vi "[ex ce]_Array - Access 1D Array elements.vi"() -> ()   [LabVIEW 2021]
doc: "<B>Example for CalcExpress script syntax</B>\n\n<B>The VI demonstrates various methods of accessing elements in 1D array</B>\n\nThis example demonstrates a use of Index Arrays and Index Ranges to perform array indexing. IndexRange feature lets you specify a sequential index subset of an array dimension. Index Array can be used to specify an arbitrary set of indeces.\n\nTo provide the Index Range feature, CalcExpress supports IndexRange Operator, IndexRange Symbols and a few IndexRange Functions. Despite they have different syntax, they have the similar functionality, so you can use any of them to specify range of indeces. In general, IndexRange symbols and functions can be convenient if you need to specify entire dimension, and IndexRange Operator can be convenient if you need to specify a sequential index subset.\n\n::: CalcExpress Toolkit :::\nCopyright (c) 2000-2026 Konstantin Shifershteyn. All rights reserved."
panel:
  in  "stop":bool
  in  "calc":bool
  in  "Expression":string
  in  "comments":string="This example demonstrates a use of Index Arrays and Index Ranges to perform array indexing. IndexRange feature lets you specify a sequential index subset of an array dimension. Index Array can be used to specify an arbitrary set of indeces.\n\nTo provide the Index Range feature, CalcExpress supports IndexRange Operator, IndexRange Symbols and a few IndexRange Functions. Despite they have different syntax, they have the similar functionality, so you can use any of them to specify range of indeces.  In general, IndexRange symbols and functions can be convenient if you need to specify entire dimension, and IndexRange Operator can be convenient if you need to specify a sequential index subset.\n"
  in  "Expressions":string[](array[string])=["idx = 5; //cell index\nlow = 2; //low boundary of Index Range\ntop = 8; //top boundary of Index Range\n\n/* cell value */\ny1 = x[idx];\n\n/* a subset in the direct order */\ny2 = x[low:top];\n\n/* a subset in the inverse order */\ny3 = x[top:low];\n\nprobe(y1, \"y1 = x[idx]\");\nprobe(y2, \"y2 = x[low:top]\");\nprobe(y3, \"y3 = x[top:low]\");\n", "y1 = y2 = y3 = y4 = x;\nidx = 1; //cell index\nlow = 2; //low boundary of Index Range\ntop = 7; //top boundary of Index Range\n\n/* assigning cell values */\ny1[idx]   = 0;\ny1[idx+1] = 1;\n\n/* assigning a subset */\ny2[low:$>] = vector(-1,-2,-3,-4);\n\n/* reversing and negating a subset */\ny3[low:top] = -y3[top:low];\n\n/* filling an array and subset */\ny4[$>] = 0;      //filling entire array\ny4[low:top] = 1; //filling a subset\n\nprobe(y1, \"y1\");\nprobe(y2, \"y2\");\nprobe(y3, \"y3\");\nprobe(y4, \"y4\");\n", "/* decimating factor */\ndf  = 2;\n\n/* step of index */\nstep = int(df);\n\n/* size of index array */\nsize = int(size(x)/step);\n\n/* creates an index array */\nidx = nvecins(0, size, step);\n\n/* get 1st decimated array */\ny1 = x[idx];\n\n/* get 2nd decimated array */\ny2 = x[idx + 1];\n\nprobe(y1, \"Decimated array 1\");\nprobe(y2, \"Decimated array 2\");\n", ""]
  in  "sel":i32(ring) items=["Obtaining indexed values", "Assigning indexed values", "Using Index Array to decimate 1D array"]
  in  "x":dbl[](array[numeric])=[100.0, 101.0, 102.0, 103.0, 104.0, 105.0, 106.0, 107.0, 108.0, 109.0] caption="(source array)" format="%.1f"
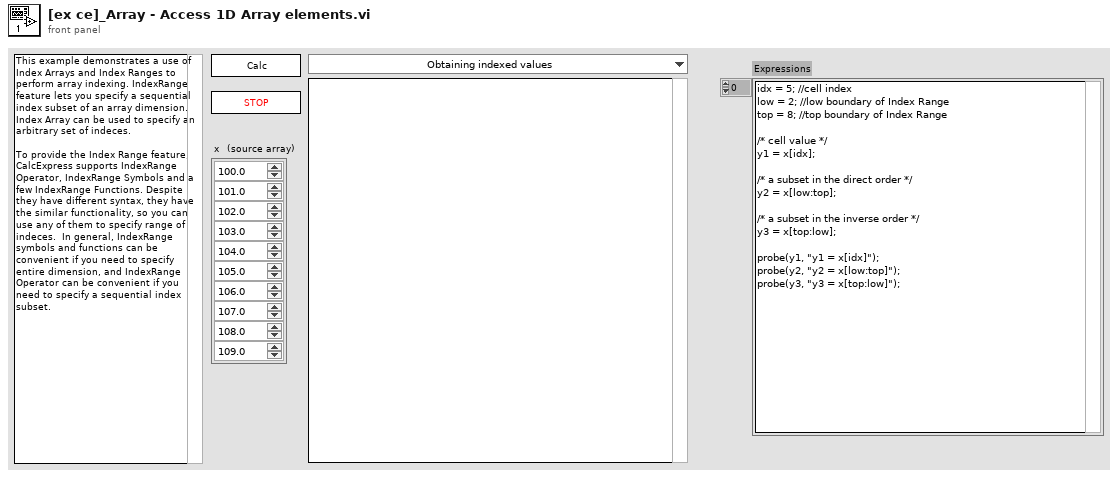
[diagram p1: front panel]
types:
  T1 = enum16{"create", "destroy", "set value", "get value"}
  T2 = typedef "VarMan Variable Context Handle.ctl" = i32
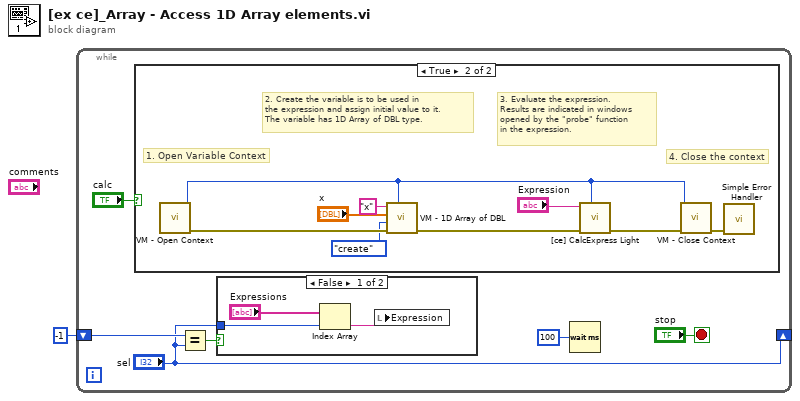
[diagram p0: block diagram]
diagram:
  n1 = while {
    shift-left: -1 ("sel") -> [w7]
    shift-right: ["sel"] -> _
    stop <- "stop" stop-if-true
    n2 = case shown="True" "calc" {
      frame False {
      }
      frame True {
        # "3. Evaluate the expression.\nResults are indicated in windows\nopened by the \"probe\" function\nin the expression."
        # "4. Close the context"
        # "2. Create the variable is to be used in\nthe expression and assign initial value to it.\nThe variable has 1D Array of DBL type."
        # "1. Open Variable Context"
        n3 = call "VM - Open Context.vi"() -> ("error out"=w19:errorcluster, "VC Handle out"=w13:T2)  [unwired: 9 in, 1 out]
        n4 = call "VM - 1D Array of DBL.vi"("VC Handle"=w13, "error in"=w19, "cmd"=T1."create", "value in"="x", "name_spec"="x" ("name")) -> ("error out"=w18:errorcluster)  [unwired: 1 in, 5 out]
        n5 = call "[ce] CalcExpress Light.vi"("VC Handle"=w13, "error in"=w18, "expression"="Expression") -> ("error out"=w12:errorcluster)  [unwired: 6 in, 2 out]
        n6 = call "VM - Close Context.vi"("error in"=w12, "VC Handle"=w13) -> ("error out"=w17:errorcluster)  [unwired: 8 in, 1 out]
        n7 = call <vilib>:"Simple Error Handler.vi"("error in (no error)"=w17) -> ()  [unwired: 4 in, 5 out]
      }
    }
    n8 = Equal?(x=w7, y="sel") -> (x = y?=w6:bool)
    n9 = case shown="False" w6 {
      tunnel: "sel" -> [w9 _]
      frame False {
        n10 = Index Array(array="Expressions", index=w9) -> (element=w8:string)
        n11 = local write "Expression"(w8) -> ()
      }
      frame True {
      }
    }
    n12 = Wait (ms)(milliseconds to wait=u32 100) -> ()  [unwired: 1 out]
  }
